vi "Initialize.vi"(8 "Error in":errorcluster caption="Error in (no error)", 9 "section postfix":string) -> (0 "Error out":errorcluster, 3 "INI-Static-Variable-Support.lvlib:CSM-Static-Variable-Manager.lvclass":refnum<class "CSM-Static-Variable-Manager.lvclass">)   [LabVIEW 2017, in "INI-Static-Variable-Support.lvlib" / "CSM-Static-Variable-Manager.lvclass"]
uses:
  CSM-Static-Variable-Manager.lvclass
  CSM-Static-Variable-Manager.lvclass/CSM-Static-Variable-Manager.ctl
  INI-Static-Variable-Support.lvlib
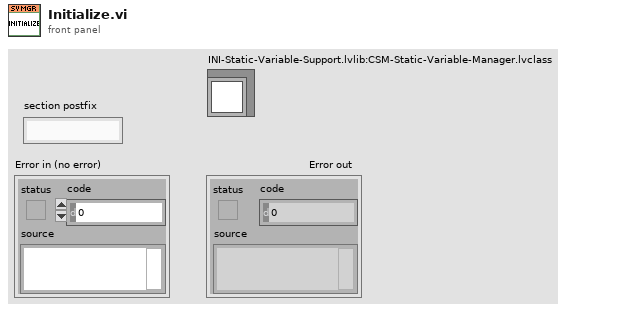
[diagram p1: front panel]
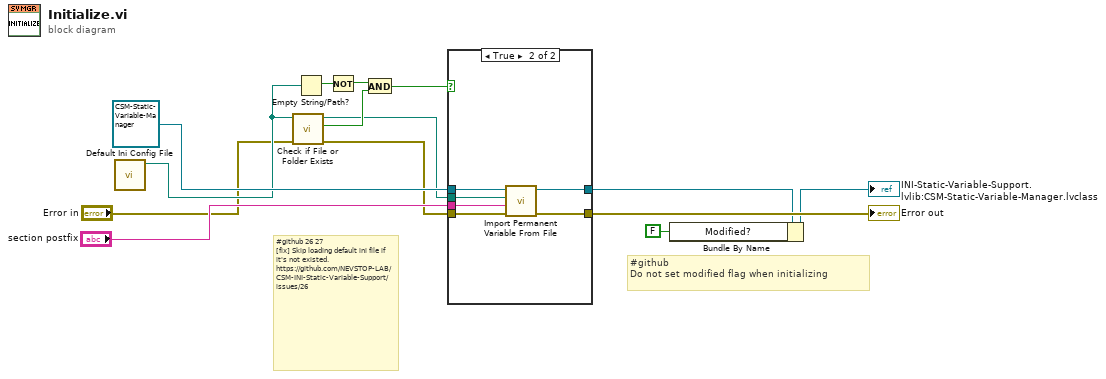
[diagram p0: block diagram]
diagram:
  # "#github\nDo not set modified flag when initializing"
  # "#github 26 27\n[fix] Skip loading default ini file if it's not existed.\nhttps://github.com/NEVSTOP-LAB/CSM-INI-Static-Variable-Support/issues/26"
  n1 = call "Default Ini Config File.vi"() -> ("appended path"=w7:path)  [unwired: 11 in]
  n2 = call <vilib>:"Check if File or Folder Exists.vi"("error in (no error)"="Error in", "path"=w7) -> ("error out"=w5:errorcluster, "file or folder exists?"=w8:bool, "dup path"=w3:path)  [unwired: 7 in]
  n3 = Empty String/Path?(string/path=w7) -> (empty?=w10:bool)
  n4 = Not(x=w10) -> (.not. x?=w9:bool)
  n5 = And(x=w9, y=w8) -> (x .and. y?=w4:bool)
  n6 = case shown="True" w4 {
    tunnel: [w15 w22] -> w14
    tunnel: refnum<class "CSM-Static-Variable-Manager.lvclass"> refnum ("INI-Static-Variable-Support.lvlib:CSM-Static-Variable-Manager.lvclass") -> [w16 w21]
    tunnel: [w16 w20] -> w12
    tunnel: "section postfix" -> [_ w19]
    tunnel: w3 -> [_ w18]
    tunnel: w5 -> [w15 w17]
    frame False {
    }
    frame True {
      n7 = call "Import Permanent Variable From File.vi"("error in (no error)"=w17, "section postfix"=w19, "Path"=w18, "CSM-Static-Variable-Manager in"=w21) -> ("error out"=w22:errorcluster, "CSM-Static-Variable-Manager out"=w20:refnum<class "CSM-Static-Variable-Manager.lvclass">)  [unwired: 6 in]
    }
  }
  "Error out" <- w14
  n8 = Bundle By Name(cluster=w12, "Modified?"=FALSE ("Memory.Modified?")) -> (→"INI-Static-Variable-Support.lvlib:CSM-Static-Variable-Manager.lvclass":refnum<class "CSM-Static-Variable-Manager.lvclass">)
